vi "Write_Frame.vi"(5 "fdf":bool, 6 "brs":bool, 7 "ide":bool, 8 "error in (no error)":errorcluster, 9 "data":u8[](array[numeric]), 10 "id":u32 format="%.0x", 11 "channel in":refnum<class "CANsub_DirectChannel.lvclass">) -> (0 "error out":errorcluster, 3 "channel out":refnum<class "CANsub_DirectChannel.lvclass">)   [LabVIEW 2021, in "CANsub_API.lvlib" / "CANsub_DirectChannel.lvclass"]
doc: "Direct: Check_Open ? W15 C_Encode_RT into the TX buffer (in place) ? Send_TX. Loop-safe: no allocation, bounded time."
uses:
  CANsub_DirectChannel.lvclass
  CANsub_DirectChannel.lvclass/CANsub_DirectChannel.ctl
  CANsub_API.lvlib
  CANsub_C.lvlib
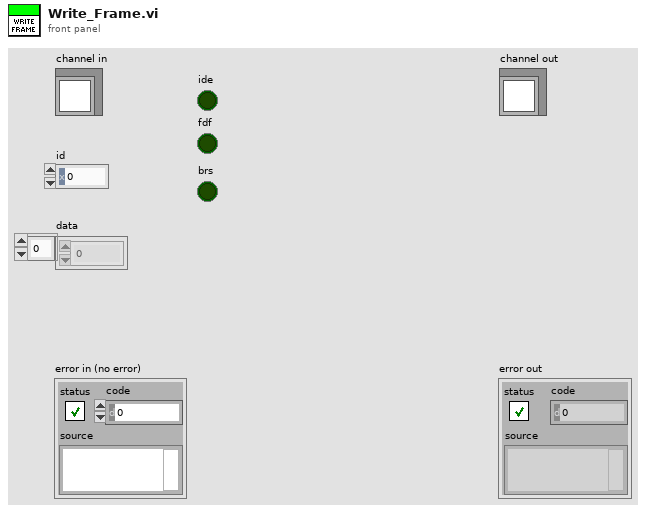
[diagram p1: front panel]
types:
  T1 = typedef "CANsub_API.lvlib/CANsub_Status.ctl" = cluster{"state":T2, "frames read":u32, "frames written":u32, "crc errors":u32, "decode errors":i32, "pings":u32, "FIFO overflows":u32, "reopens":u32, "nodelay":i32, "api version":string, "lib version":u32, "bit timing":T3, "last error":errorcluster}
  T2 = typedef "CANsub_API.lvlib/CANsub_State.ctl" = enum16{"Closed", "Open", "Lost"}
  T3 = typedef "CANsub_Common.lvlib/Bit_Timing.ctl" = cluster{"brp":u16, "seg1":u16, "seg2":u16, "sjw":u16, "data brp":u16, "data seg1":u16, "data seg2":u16, "data sjw":u16}
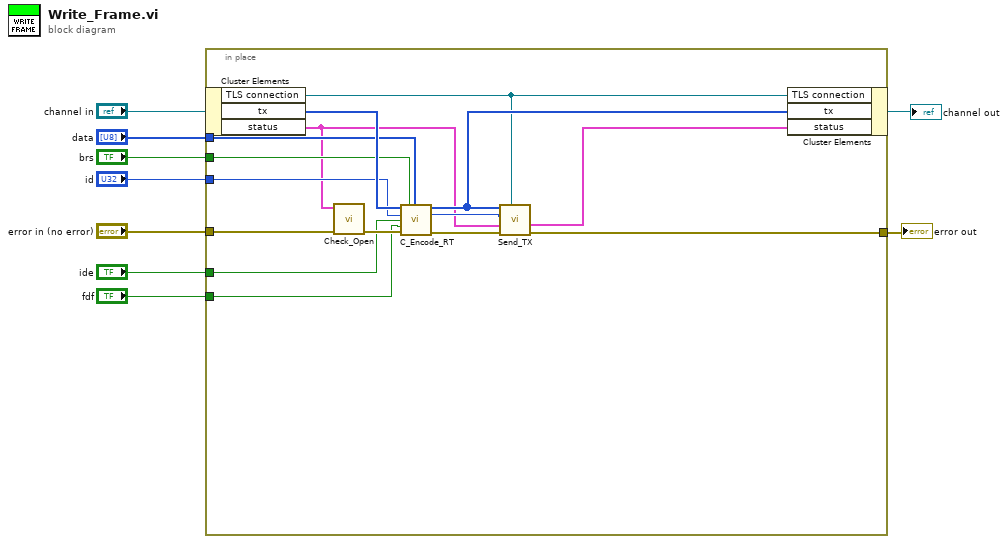
[diagram p0: block diagram]
diagram:
  n1 = in-place {
    in-place-border: "error in (no error)" -> [w24]
    in-place-border: "brs" -> [w21]
    in-place-border: "id" -> [w20]
    in-place-border: "ide" -> [w19]
    in-place-border: "fdf" -> [w18]
    in-place-border: "data" -> [w17]
    in-place-border: [w10] -> w1
    n2 = in-place-cluster #1("channel in") -> ("TLS connection"=w15:refnum<k5>, "tx"=w22:u8[], "status"=w13:T1)
    n3 = call "Check_Open.vi"("error in (no error)"=w24, "status"=w13) -> ("error out"=w23:errorcluster)  [unwired: 9 in]
    n4 = call "C_Encode_RT.vi"("tx in"=w22, "brs"=w21, "data"=w17, "id"=w20, "ide"=w19, "fdf"=w18, "error in (no error)"=w23) -> ("tx out"=w16:u8[], "length"=w14:i32, "error out"=w11:errorcluster)  [unwired: 6 in]
    n5 = call "Send_TX.vi"("TLS connection"=w15, "error in (no error)"=w11, "status in"=w13, "length"=w14, "tx"=w16) -> ("error out"=w10:errorcluster, "status out"=w12:T1)  [unwired: 5 in]
    n6 = in-place-cluster #1("TLS connection"=w15, "tx"=w16, "status"=w12) -> (→"channel out":refnum<class "CANsub_DirectChannel.lvclass">)
  }
  "error out" <- w1
